vi "Read Message.vi"(8 "error in (no error)":errorcluster, 11 "RemoteControl.ZMQ in":refnum<class "RemoteControl.ZMQ.lvclass">) -> (0 "error out":errorcluster, 2 "Message":T1, 3 "RemoteControl.ZMQ out":refnum<class "RemoteControl.ZMQ.lvclass">)   [LabVIEW 2019, in "RemoteControl.ZMQ.lvlib" / "RemoteControl.ZMQ.lvclass"]
uses:
  RemoteControl.ZMQ.lvclass
  C:/Program Files/National Instruments/LabVIEW 2019/user.lib/LevyLab/RemoteControl/RemoteControl/RemoteControl.lvclass
  <userlib>/LevyLab/RemoteControl/RemoteControl/Typedefs/Message--Cluster.ctl
  <userlib>/LevyLab/RemoteControl/RemoteControl/RemoteControl.lvclass/RemoteControl.ctl
  RemoteControl.ZMQ.lvclass/RemoteControl.ZMQ.ctl
  <vilib>/Utility/error.llb/Error Cluster From Error Code.vi
  <vilib>/ErrorRing/Error Ring.xnode
  <vilib>/PRIrvin/JSON-RPC/JSON-RPC.lvlib
  <vilib>/addons/zeromq/zmq_socket.lvclass
  <userlib>/LevyLab/RemoteControl/RemoteControl/RemoteControl.lvclass
  C:/Program Files/National Instruments/LabVIEW 2019/vi.lib/JKI/JKI SMO/SMO/SMO.lvclass
panel:
  out "Retry#":i32
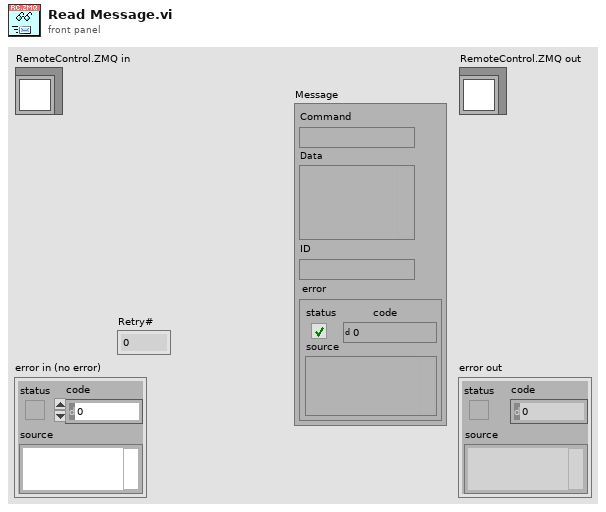
[diagram p1: front panel]
types:
  T1 = typedef "RemoteControl.lvlib/RemoteControl.lvclass/Message--Cluster.ctl" = cluster{"Command":string, "Data":variant, "ID":string, "error":errorcluster}
  T2 = typedef "zeromq.lvlib/socket_type.ctl" = enum8{"ZMQ_PAIR", "ZMQ_PUB", "ZMQ_SUB", "ZMQ_REQ", "ZMQ_REP", "ZMQ_DEALER", "ZMQ_ROUTER", "ZMQ_PULL", "ZMQ_PUSH", "ZMQ_XPUB", "ZMQ_XSUB", "ZMQ_STREAM", "ZMQ_SERVER", "ZMQ_CLIENT", "ZMQ_RADIO", "ZMQ_DISH", "ZMQ_GATHER", "ZMQ_SCATTER", "ZMQ_DGRAM"}
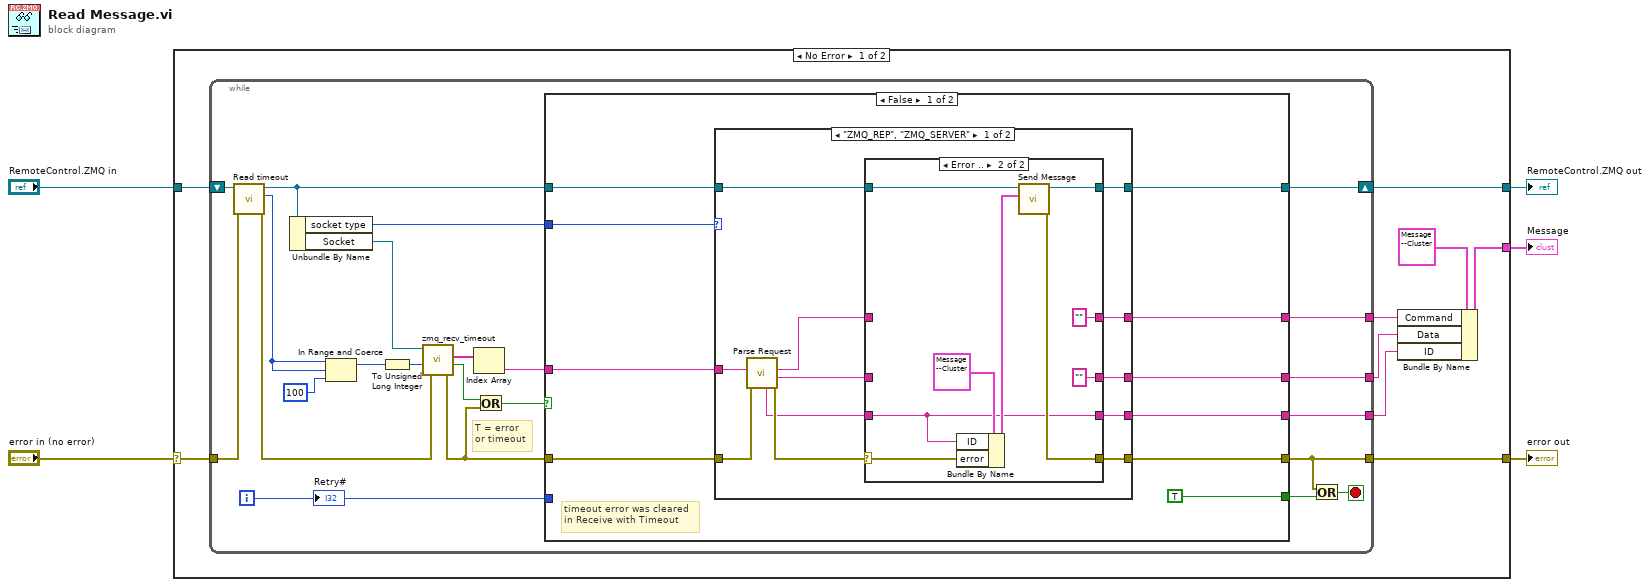
[diagram p0: block diagram]
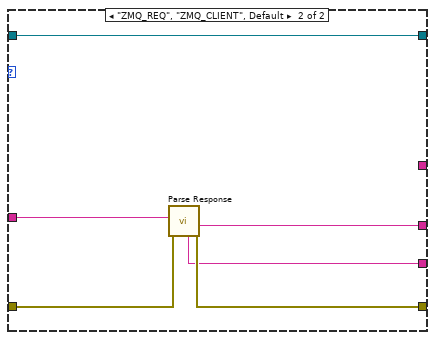
[diagram p3: hidden frame]
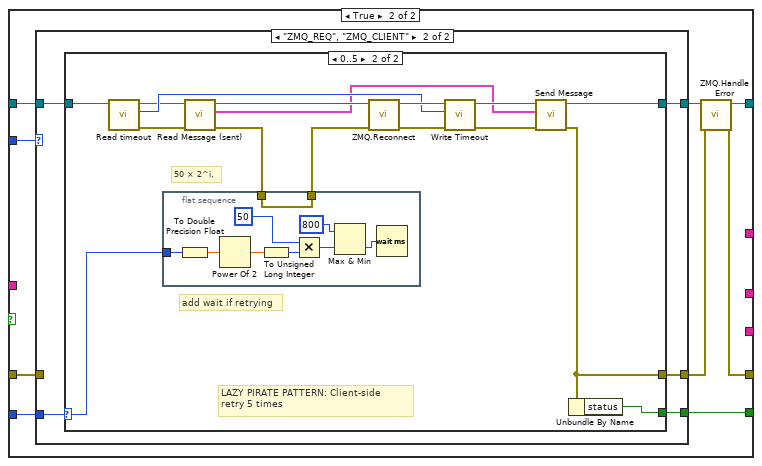
[diagram p4: hidden frame]
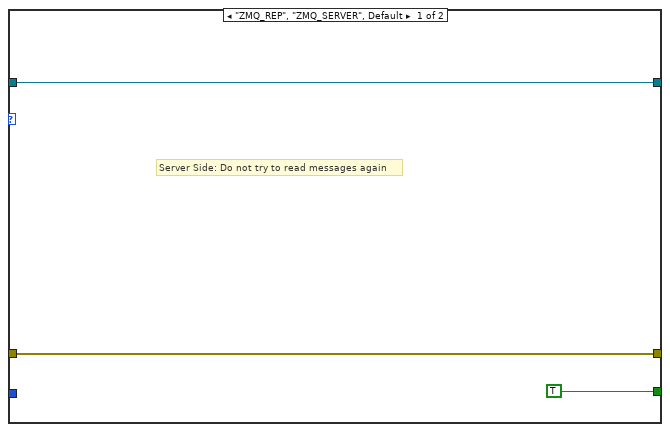
[diagram p5: hidden frame]
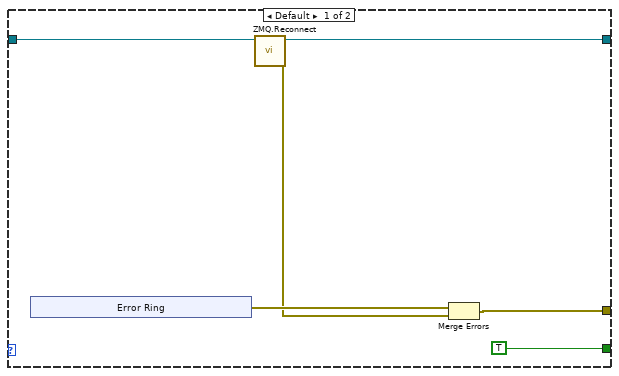
[diagram p6: hidden frame]
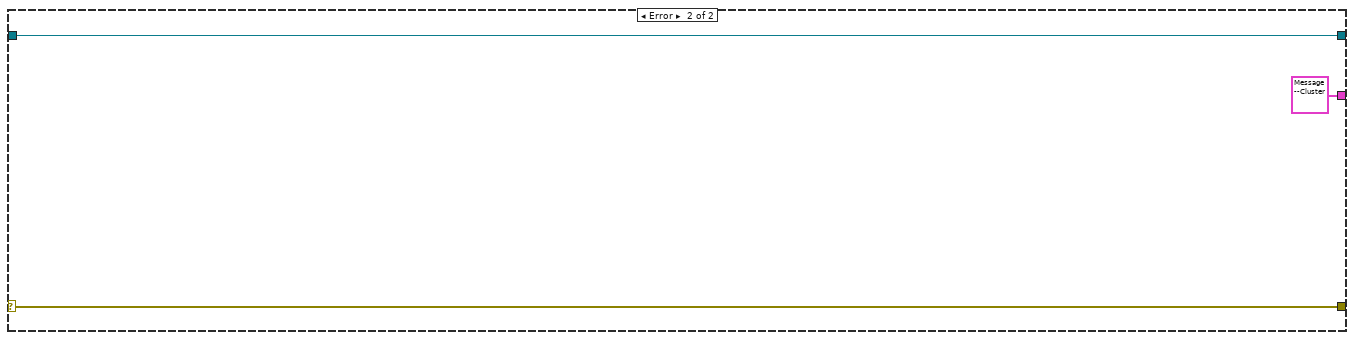
[diagram p7: hidden frame]
diagram:
  n1 = case shown="No Error" "error in (no error)" {
    selector: "error in (no error)" -> [w11 w134]
    tunnel: [w14 w134] -> w5
    tunnel: [w13 w133] -> w4
    tunnel: "RemoteControl.ZMQ in" -> [w12 w133]
    tunnel: [w9 T1 {"Command"="", "Data"=variant, "ID"="", "error"={"status"=FALSE, "code"=0, "source"=""}} ("Message")] -> w1
    frame No Error {
      n2 = while {
        tunnel: [w37] -> w8
        tunnel: [w36] -> w7
        tunnel: [w35] -> w6
        tunnel: w11 -> [w25]
        tunnel: [w28] -> w14
        shift-right: [w27] -> w13
        shift-left: w12 -> [w26]
        i -> [w32]
        stop <- w34 stop-if-true
        # "T = error\nor timeout"
        n3 = call <userlib>:"Read timeout.vi"("error in (no error)"=w25, "RemoteControl in"=w26) -> ("error out"=w20:errorcluster, "timeout"=w16:i32, "RemoteControl out"=w29:refnum<class "RemoteControl.ZMQ.lvclass">)  [unwired: 7 in]
        n4 = Unbundle By Name(w29) -> ("socket type"=w24:T2, "Socket"=w21:refnum<class "zmq_socket.lvclass">)
        n5 = In Range and Coerce(upper limit=w16, x=w16, lower limit=100) -> (coerced(x)=w15:i32)  [unwired: 1 out]
        n6 = To Unsigned Long Integer(number=w15) -> (unsigned 32bit integer=w22:u32)
        n7 = call <vilib>:"zmq_recv_timeout.vi"("error in"=w20, "timeout (ms)"=w22, "socket in"=w21) -> ("error out"=w19:errorcluster, "timeout?"=w18:bool, "parts"=w23:string[])  [unwired: 1 in, 1 out]
        n8 = Index Array(array=w23) -> (element=w31:string)  [unwired: 1 in]
        n9 = Or(x=w18, y=w19) -> (x .or. y?=w30:bool)
        n10 = case shown="False" w30 {
          tunnel: [w47 _] -> w36
          tunnel: [w46 _] -> w35
          tunnel: [w45 _] -> w37
          tunnel: w24 -> [w40 w87]
          tunnel: w29 -> [w39 w88]
          tunnel: [w38 w80] -> w27
          tunnel: w32 -> [_ w86]
          tunnel: [w44 w81] -> w28
          tunnel: [TRUE w85] -> w33
          tunnel: w19 -> [w43 w84]
          tunnel: w31 -> [w41 _]
          frame False {
            # "timeout error was cleared\nin Receive with Timeout"
            n11 = case shown="\"ZMQ_REP\", \"ZMQ_SERVER\"" w40 {
              tunnel: w41 -> [w58 w76]
              tunnel: w43 -> [w59 w79]
              tunnel: [w53 w78] -> w44
              tunnel: [w50 _] -> w45
              tunnel: [w48 w75] -> w47
              tunnel: [w52 w77] -> w46
              tunnel: w39 -> [w55 w74]
              tunnel: [w54 w74] -> w38
              frame "ZMQ_REP", "ZMQ_SERVER" {
                n12 = call <vilib>:"Parse Request.vi"("error in (no error)"=w59, "<JSON> Requests"=w58) -> ("error out"=w57:errorcluster, "Params"=w49:string, "Methods"=w51:string, "IDs"=w56:string)  [unwired: 6 in]
                n13 = case shown="Error .." w57 {
                  selector: w57 -> [w63 w67]
                  tunnel: w56 -> [w62 w65]
                  tunnel: w55 -> [w64 w70]
                  tunnel: [w64 w71] -> w54
                  tunnel: [w63 w69] -> w53
                  tunnel: [w62 w65] -> w52
                  tunnel: w51 -> [w61 _]
                  tunnel: [w61 "" ("Methods")] -> w50
                  tunnel: w49 -> [w60 _]
                  tunnel: [w60 "" ("Params")] -> w48
                  frame No Error {
                  }
                  frame Error {
                    n14 = Bundle By Name(cluster=T1 {"Command"="", "Data"=variant, "ID"="", "error"={"status"=FALSE, "code"=0, "source"=""}} ("Message"), "ID"=w65, "error"=w67) -> (w66:T1)
                    n15 = call-dynamic "Send Message.vi"("Message"=w66, "RemoteControl.ZMQ in"=w70) -> ("error out"=w69:errorcluster, "RemoteControl.ZMQ out"=w71:refnum<class "RemoteControl.ZMQ.lvclass">)  [unwired: 8 in]
                  }
                }
              }
              frame "ZMQ_REQ", "ZMQ_CLIENT", Default {
                n16 = call <vilib>:"Parse Response.vi"("error in (no error)"=w79, "<JSON> Response"=w76) -> ("error out"=w78:errorcluster, "results"=w75:string, "IDs"=w77:string)  [unwired: 7 in]
              }
            }
          }
          frame True {
            n17 = case shown="\"ZMQ_REQ\", \"ZMQ_CLIENT\"" w87 {
              tunnel: w88 -> [w91 w96]
              tunnel: [w91 w95] -> w83
              tunnel: w86 -> [_ w92]
              tunnel: [w90 w94] -> w82
              tunnel: [TRUE w93] -> w85
              tunnel: w84 -> [w90 _]
              frame "ZMQ_REP", "ZMQ_SERVER", Default {
                # "Server Side: Do not try to read messages again"
              }
              frame "ZMQ_REQ", "ZMQ_CLIENT" {
                n18 = case shown="0..5" w92 {
                  selector: w92 -> [_ w112]
                  tunnel: w96 -> [w100 w121]
                  tunnel: [w101 w122] -> w95
                  tunnel: [w98 w107] -> w94
                  tunnel: [TRUE w108] -> w93
                  frame Default {
                    n19 = xnode "Error Ring"() -> ("error out"=w99:errorcluster)
                    n20 = call "ZMQ.Reconnect.vi"("RemoteControl.ZMQ in"=w100) -> ("error out"=w97:errorcluster, "RemoteControl.ZMQ out"=w101:refnum<class "RemoteControl.ZMQ.lvclass">)  [unwired: 9 in]
                    n21 = Merge Errors(w99, w97) -> (w98:errorcluster)
                  }
                  frame 0..5 {
                    # "add wait if retrying"
                    # "50 × 2^i,"
                    # "LAZY PIRATE PATTERN: Client-side\nretry 5 times"
                    n22 = call <userlib>:"Read timeout.vi"("RemoteControl in"=w121) -> ("error out"=w117:errorcluster, "timeout"=w118:i32, "RemoteControl out"=w116:refnum<class "RemoteControl.ZMQ.lvclass">)  [unwired: 8 in]
                    n23 = flat-sequence {
                      tunnel: w112 -> [w127]
                      tunnel: [w126] -> w111
                      tunnel: w110 -> [w126]
                      frame #0 {
                        n24 = To Double Precision Float(number=w127) -> (double precision float=w128:dbl)
                        n25 = Power Of 2(x=w128) -> (2^x=w131:dbl)
                        n26 = To Unsigned Long Integer(number=w131) -> (unsigned 32bit integer=w129:u32)
                        n27 = Multiply(x=u32 50 ("milliseconds to wait"), y=w129) -> (x*y=w125:u32)
                        n28 = Max & Min(x=u32 800 ("upper limit"), y=w125) -> (min(x,y)=w123:u32)  [unwired: 1 out]
                        n29 = Wait (ms)(milliseconds to wait=w123) -> ()  [unwired: 1 out]
                      }
                    }
                    n30 = call <userlib>:"Read Message (sent).vi"("error in (no error)"=w117, "RemoteControl in"=w116) -> ("error out"=w110:errorcluster, "Message (sent)"=w109:T1, "RemoteControl out"=w115:refnum<class "RemoteControl.ZMQ.lvclass">)  [unwired: 7 in]
                    n31 = call "ZMQ.Reconnect.vi"("error in (no error)"=w111, "RemoteControl.ZMQ in"=w115) -> ("error out"=w119:errorcluster, "RemoteControl.ZMQ out"=w120:refnum<class "RemoteControl.ZMQ.lvclass">)  [unwired: 8 in]
                    n32 = call <userlib>:"Write Timeout.vi"("error in (no error)"=w119, "timeout (ms) [500]"=w118, "RemoteControl in"=w120) -> ("error out"=w113:errorcluster, "RemoteControl out"=w114:refnum<class "RemoteControl.ZMQ.lvclass">)  [unwired: 7 in]
                    n33 = call-dynamic "Send Message.vi"("error in (no error)"=w113, "Message"=w109, "RemoteControl.ZMQ in"=w114) -> ("error out"=w107:errorcluster, "RemoteControl.ZMQ out"=w122:refnum<class "RemoteControl.ZMQ.lvclass">)  [unwired: 7 in]
                    n34 = Unbundle By Name(w107) -> ("status"=w108:bool)
                  }
                }
              }
            }
            n35 = call "ZMQ.Handle Error.vi"("error in (no error)"=w82, "RemoteControl.ZMQ in"=w83) -> ("error out"=w81:errorcluster, "RemoteControl.ZMQ out"=w80:refnum<class "RemoteControl.ZMQ.lvclass">)  [unwired: 8 in]
          }
        }
        n36 = Or(x=w28, y=w33) -> (x .or. y?=w34:bool)
        "Retry#" <- w32
      }
      n37 = Bundle By Name(cluster=T1 {"Command"="", "Data"=variant, "ID"="", "error"={"status"=FALSE, "code"=0, "source"=""}} ("Message"), "Command"=w8, "Data"=w7, "ID"=w6) -> (w9:T1)
    }
    frame Error {
    }
  }
  "error out" <- w5
  "RemoteControl.ZMQ out" <- w4
  "Message" <- w1
